vi "set Measurement Window Mode - FSV40.vi"(8 "error in (no error)":errorcluster, 10 "Measurement Window Mode":T1, 11 "FSV-40N in":refnum<class "FSV-40N.lvclass">) -> (0 "error out":errorcluster, 3 "FSV-40N out":refnum<class "FSV-40N.lvclass">)   [LabVIEW 2023, in "Spectrum Analyzer.lvlib" / "FSV-40N.lvclass"]
doc: "1) ACPower\nAdjacent-channel power measurement with a single carrier signal\n2) CPOWer\nChannel power measurement with a single carrier signal (equivalent to adjacent-channel power measurement with \"NO. OF ADJ CHAN\" = 0)\n3) MCACpower\nChannel/adjacent-channel power measurement with several carrier signals\n4) OBANdwidth | OBWidth\nMeasurement of occupied bandwidth\n5) CN\nMeasurement of carrier-to-noise ratio\n6) CN0\nMeasurement of carrier-to-noise ratio referenced to 1 Hz bandwidth"
uses:
  FSV-40N.lvclass
  TYPE DEFINITION/TYPE Measurement Window Mode.ctl
  FSV-40N.lvclass/FSV-40N.ctl
  Spectrum Analyzer.lvlib
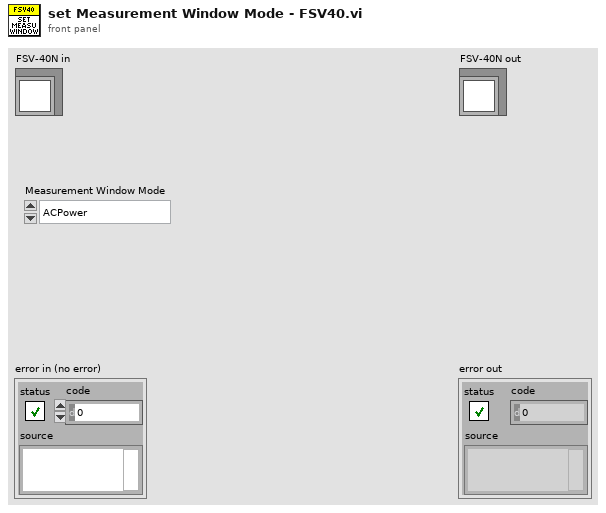
[diagram p1: front panel]
types:
  T1 = typedef "Spectrum Analyzer.lvlib/TYPE Measurement Window Mode.ctl" = enum16{"ACPower", "CPOWer", "MCACpower", "OBANdwidth", "OBWidth", "CN", "CN0"}
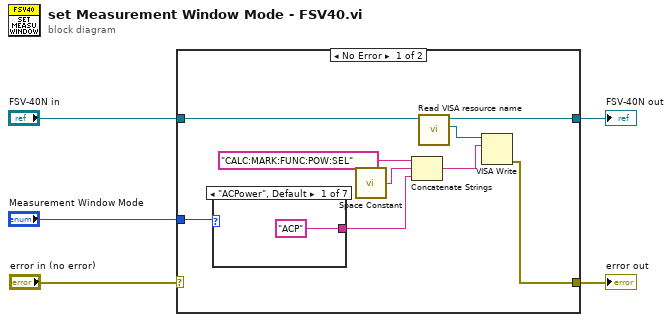
[diagram p0: block diagram]
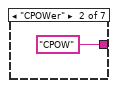
[diagram p2: hidden frame]
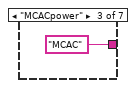
[diagram p3: hidden frame]
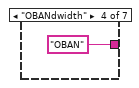
[diagram p4: hidden frame]
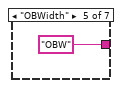
[diagram p5: hidden frame]
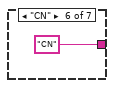
[diagram p6: hidden frame]
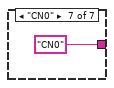
[diagram p7: hidden frame]
diagram:
  n1 = case shown="No Error" "error in (no error)" {
    selector: "error in (no error)" -> [_ w22]
    tunnel: "FSV-40N in" -> [w14 w23]
    tunnel: [w7 w23] -> w3
    tunnel: [w6 w22] -> w2
    tunnel: "Measurement Window Mode" -> [w13 _]
    frame No Error {
      n2 = case shown="\"ACPower\", Default" w13 {
        tunnel: ["ACP" "CPOW" "MCAC" "OBAN" "OBW" "CN" "CN0"] -> w10
        frame "ACPower", Default {
        }
        frame "CPOWer" {
        }
        frame "MCACpower" {
        }
        frame "OBANdwidth" {
        }
        frame "OBWidth" {
        }
        frame "CN" {
        }
        frame "CN0" {
        }
      }
      n3 = call <vilib>:"Space Constant.vi"() -> ("String"=w11:string)
      n4 = Concatenate Strings("CALC:MARK:FUNC:POW:SEL" ("string"), w11, w10) -> (w8:string)
      n5 = call "Read VISA resource name.vi"("FSV-40N in"=w14) -> ("VISA resource name"=w9:refnum<visa-resource-name>, "FSV-40N out"=w7:refnum<class "FSV-40N.lvclass">)  [unwired: 8 in, 1 out]
      n6 = VISA Write(VISA resource name=w9, write buffer=w8) -> (error out=w6:errorcluster)  [unwired: 1 in, 2 out]
    }
    frame Error {
    }
  }
  "error out" <- w2
  "FSV-40N out" <- w3
